vi "Get CD Storage Library Loader Ref.vi"(11 "DMA Channel Testing in":refnum<class "FPGA Addon DMA Channel Unit Tests.lvclass">) -> (2 "CDS Loader Ref":refnum<vi>, 3 "DMA Channel Testing out":refnum<class "FPGA Addon DMA Channel Unit Tests.lvclass">)   [LabVIEW 2020, in "FPGA Addon DMA Channel Unit Tests.lvclass"]
uses:
  FPGA Addon DMA Channel Unit Tests.lvclass
  FPGA Addon DMA Channel Unit Tests.lvclass/FPGA Addon DMA Channel Unit Tests.ctl
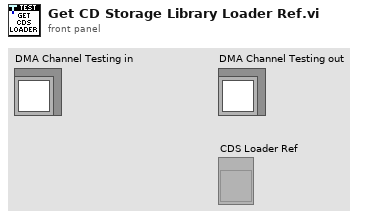
[diagram p1: front panel]
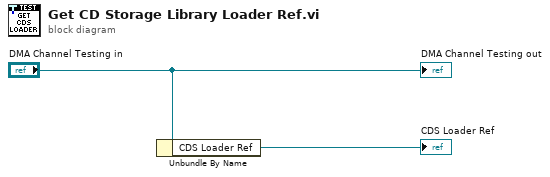
[diagram p0: block diagram]
diagram:
  n1 = Unbundle By Name("DMA Channel Testing in") -> ("CDS Loader Ref"=→"CDS Loader Ref":refnum<vi>)
  "DMA Channel Testing out" <- "DMA Channel Testing in"
